vi "Write Text.vi"(8 "error in (no error)":errorcluster, 9 "timeout ms (5000)":i32=5000, 10 "String Data":string, 11 "WebSocket in":refnum<class "WebSocket.lvclass">) -> (0 "error out":errorcluster, 3 "WebSocket out":refnum<class "WebSocket.lvclass">)   [LabVIEW 2013, in "WebSockets.lvlib" / "WebSocket.lvclass"]
doc: "Writes a text frame to the WebSocket connection endpoint."
uses:
  WebSocket.lvclass
  Opcodes.ctl
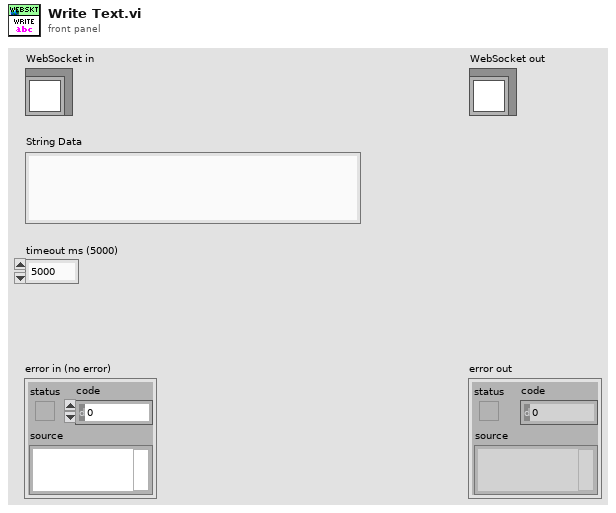
[diagram p1: front panel]
types:
  T1 = typedef "WebSockets.lvlib/WebSocket.lvclass/Opcodes.ctl" = u8
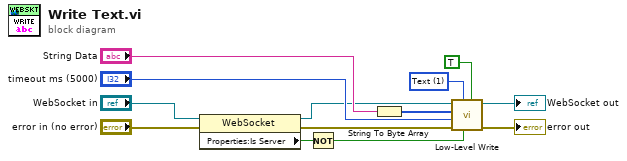
[diagram p0: block diagram]
diagram:
  w8 = T1 1 items=["Cont. Frame"=0, "Text"=1, "Binary"=2, "Close Frame"=8, "Ping"=9, "Pong"=10] ("Opcode (Text)")
  n1 = property class="WebSocket"(reference="WebSocket in", error in="error in (no error)") -> (reference out=w5:refnum<class "WebSocket.lvclass">, error out=w3:errorcluster, "Properties:Is Server"=w2:bool)
  n2 = Not(x=w2) -> (.not. x?=w1:bool)
  n3 = String To Byte Array(string="String Data") -> (unsigned byte array=w7:u8[])
  n4 = call "Low-Level Write.vi"("Finished? (True)"=TRUE, "Mask payload?"=w1, "Opcode (Text)"=w8, "error in (no error)"=w3, "timeout ms (5000)"="timeout ms (5000)", "Data"=w7, "WebSockets in"=w5) -> ("error out"=→"error out":errorcluster, "WebSockets out"=→"WebSocket out":refnum<class "WebSocket.lvclass">)  [unwired: 3 in]
